vi "Timer_Create.vi"(8 "error in (no error)":errorcluster={"status"=FALSE, "code"=0, "source"="\"\""}, 10 "duration":string, 11 "Timer purpose":string) -> (0 "error out":errorcluster={"status"=FALSE, "code"=0, "source"="\"\""}, 2 "status ok":bool, 3 "TimerTicket":string)   [LabVIEW 2026]
doc: "INTENT: Register a nonblocking deadline. LOGIC: Compute monotonic deadline and scope (ACK/feedback/stabilize/dwell/capture)."
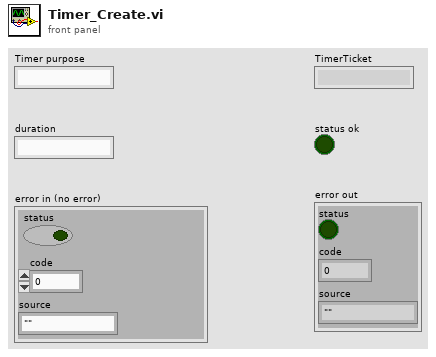
[diagram p1: front panel]
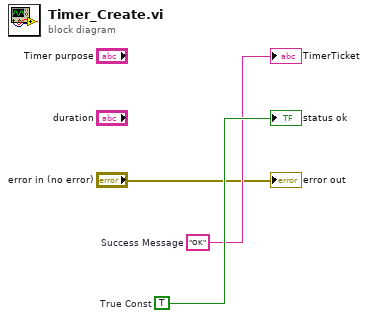
[diagram p0: block diagram]
diagram:
  w3 = TRUE  # True Const
  w2 = "OK"  # Success Message
  "TimerTicket" <- w2
  "status ok" <- w3
  "error out" <- "error in (no error)"
